vi "GO alerte min-max temperatures.vi"(3 "Numéro":u8) -> (0 "défaut températures min/max":bool)   [LabVIEW 2022 SP3]
uses:
  Enum/Enum s1.ctl
  Variables globales/Variable glob alertes min-max temperatures.vi
  Variables globales/Variable glob mails.vi
  Variables globales/Variables glob EUROTHERM.vi
  Variables globales/Variable glob Th.vi
  Variables globales/Variable glob generale.vi
  Variables globales/Variable glob Pt.vi
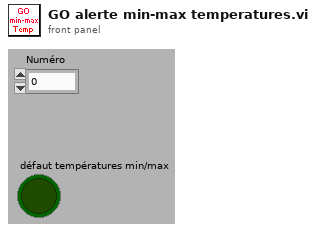
[diagram p1: front panel]
types:
  T1 = typedef "Enum s1.ctl" = enum16{"Alerte vide", "Alerte temperature min-max", "Alerte temperature ecart", "Alerte Keller", "Alerte compteur", "Alerte régulateurs"}
  T2 = cluster{"Alerte temp min/max":bool, "température max":dbl, "température min":dbl, "Défaut min/max temp":bool, "Indices à controler":i16[], "N°":u16}[]
  T3 = cluster{"Alerte temp min/max":bool, "température max":dbl, "température min":dbl, "Défaut min/max temp":bool, "Indices à controler":i16[], "N°":u16}
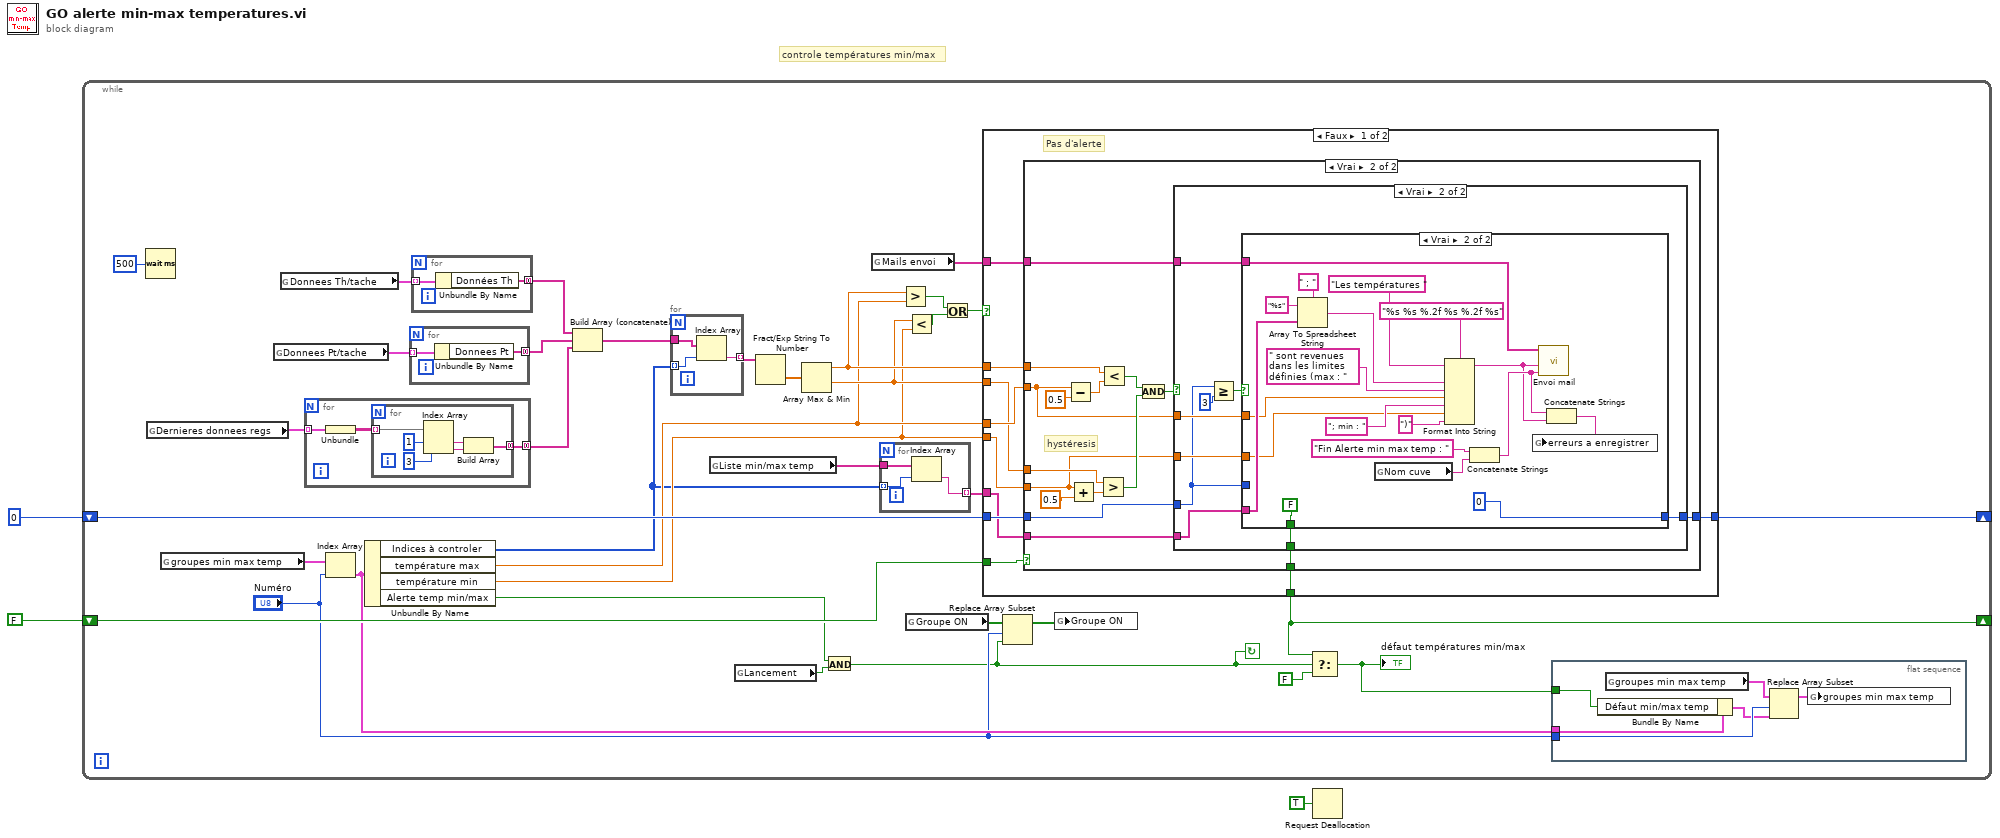
[diagram p0: block diagram]
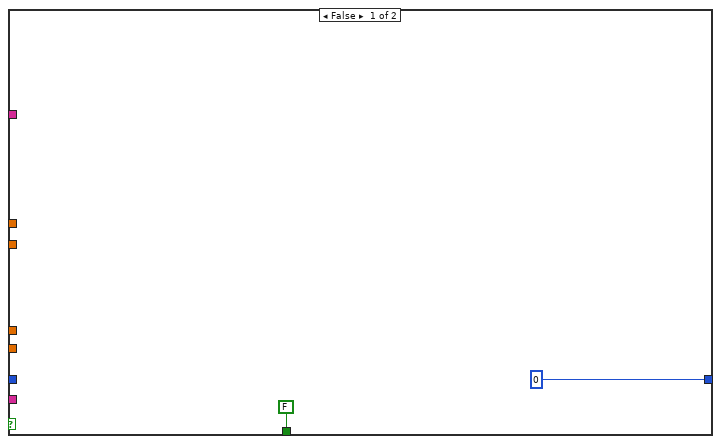
[diagram p2: hidden frame]
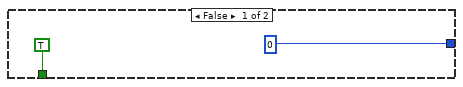
[diagram p3: hidden frame]
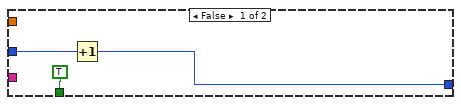
[diagram p4: hidden frame]
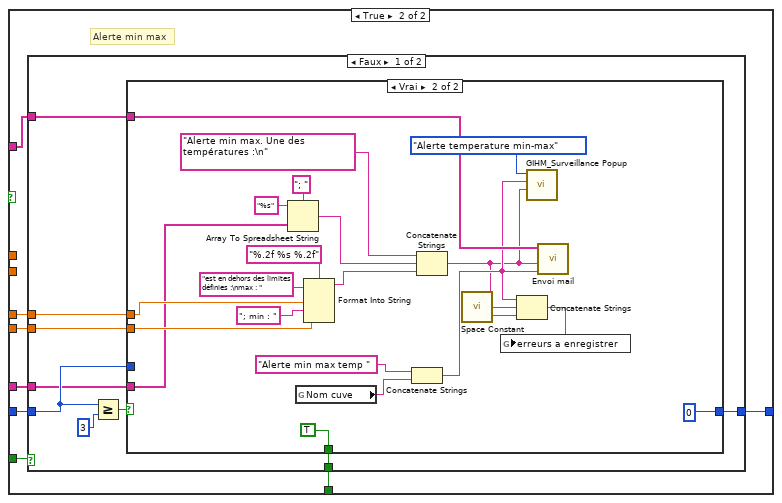
[diagram p5: hidden frame]
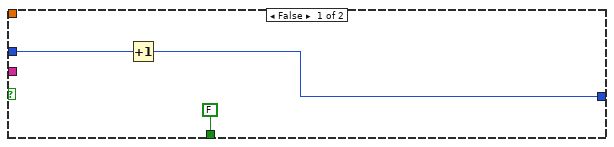
[diagram p6: hidden frame]
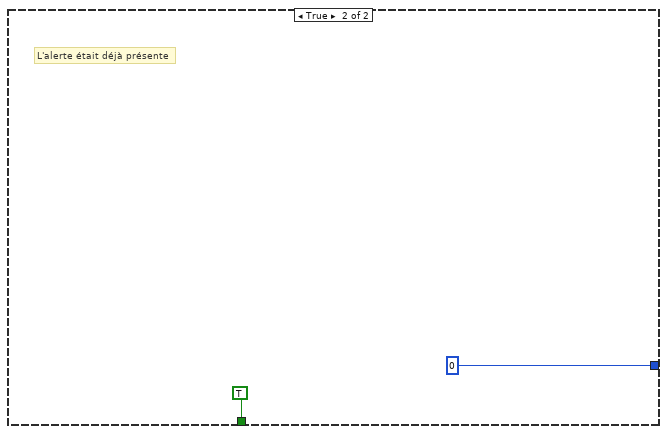
[diagram p7: hidden frame]
diagram:
  # "controle températures min/max"
  n1 = while {
    shift-right: [w22] -> _
    shift-left: FALSE -> [w35]
    shift-right: [w27] -> _
    shift-left: 0 -> [w28]
    stop <- w4 continue-if-true
    n2 = Wait (ms)(milliseconds to wait=u32 500 ("attente (ms)")) -> ()  [unwired: 1 out]
    n3 = global read "Variables glob EUROTHERM.vi" "Dernieres donnees regs"() -> (w18:cluster{"Dernieres donnees 1COM":string[][]}[])
    n4 = global read "Variable glob alertes min-max temperatures.vi" "groupes min max temp"() -> (w13:T2)
    n5 = global read "Variable glob Pt.vi" "Donnees Pt/tache"() -> (w24:cluster{"Donnees Pt":string[]}[])
    n6 = global read "Variable glob Th.vi" "Donnees Th/tache"() -> (w26:cluster{"Données Th":string[]}[])
    n7 = for {
      tunnel: w18 -> [w50] mode=indexing
      tunnel: [w48] -> w17 mode=concatenating
      n8 = Unbundle(w50) -> ("Dernieres donnees 1COM"=w49:string[][])
      n9 = for {
        tunnel: w49 -> [w56] mode=indexing
        tunnel: [w51] -> w48 mode=concatenating
        n10 = Index Array(array=w56, index #1=1 ("indice"), index #2=3 ("longueur")) -> (element #1=w53:string, element #2=w52:string)
        n11 = Build Array(w53, w52) -> (w51:string[])
      }
    }
    n12 = Index Array(array=w13, index="Numéro") -> (element=w15:T3)
    n13 = Unbundle By Name(w15) -> ("Indices à controler"=w12:i16[], "température max"=w20:dbl, "température min"=w19:dbl, "Alerte temp min/max"=w9:bool)
    n14 = for {
      tunnel: w24 -> [w58] mode=indexing
      tunnel: [w57] -> w23 mode=concatenating
      n15 = Unbundle By Name(w58) -> ("Donnees Pt"=w57:string[])
    }
    n16 = for {
      tunnel: w26 -> [w60] mode=indexing
      tunnel: [w59] -> w25 mode=concatenating
      n17 = Unbundle By Name(w60) -> ("Données Th"=w59:string[])
    }
    n18 = Build Array (concatenate)(w25, w23, w17) -> (w31:string[])
    n19 = for {
      tunnel: w31 -> [w166]
      tunnel: w12 -> [w167] mode=indexing
      tunnel: [w165] -> w38 mode=indexing
      n20 = Index Array(array=w166, index=w167) -> (element=w165:string)
    }
    n21 = global read "Variable glob alertes min-max temperatures.vi" "Liste min/max temp"() -> (w11:string[])
    n22 = global read "Variable glob generale.vi" "Lancement"() -> (w33:bool)
    n23 = Fract/Exp String To Number(string=w38) -> (number=w34:dbl[])  [unwired: 3 in, 1 out]
    n24 = Array Max & Min(array=w34) -> (max value=w30:dbl, min value=w29:dbl)  [unwired: 2 out]
    n25 = And(x=w9, y=w33) -> (x .and. y?=w4:bool)
    n26 = global read "Variable glob mails.vi" "Mails envoi"() -> (w8:string[])
    n27 = for {
      tunnel: w12 -> [w46] mode=indexing
      tunnel: w11 -> [w47]
      tunnel: [w45] -> w10 mode=indexing
      n28 = Index Array(array=w47, index=w46) -> (element=w45:string)
    }
    n29 = Greater?(x=w30, y=w20) -> (0:w36:bool)
    n30 = global read "Variable glob alertes min-max temperatures.vi" "Groupe ON"() -> (w7:bool[])
    n31 = Less?(x=w29, y=w19) -> (x < y?=w37:bool)
    n32 = Or(x=w36, y=w37) -> (x .or. y?=w32:bool)
    n33 = case shown="Faux" w32 {
      tunnel: w35 -> [w70 w129]
      tunnel: w8 -> [w69 w128]
      tunnel: w30 -> [w68 _]
      tunnel: w20 -> [w67 w125]
      tunnel: w29 -> [w66 _]
      tunnel: w19 -> [w65 w126]
      tunnel: [w64 w127] -> w22
      tunnel: w28 -> [w63 w124]
      tunnel: [w62 w123] -> w27
      tunnel: w10 -> [w61 w122]
      frame False {
        # "Pas d'alerte"
        # "Pas ou plus d'alerte"
        n34 = case shown="Vrai" w70 {
          tunnel: w69 -> [_ w88]
          tunnel: w68 -> [_ w81]
          tunnel: w67 -> [_ w79]
          tunnel: w66 -> [_ w84]
          tunnel: w65 -> [_ w78]
          tunnel: [FALSE w76] -> w64
          tunnel: w63 -> [_ w74]
          tunnel: [0 w75] -> w62
          tunnel: w61 -> [_ w73]
          frame False {
            # "Il n'y avait pas d'alerte la fois précédente"
          }
          frame True {
            # "hystéresis"
            # "Il y avait une alerte la fois précédente"
            n35 = Subtract(x=w79, y=0.5) -> (x-y=w80:dbl)
            n36 = Add(x=w78, y=0.5) -> (x+y=w85:dbl)
            n37 = Greater?(x=w84, y=w85) -> (0:w82:bool)
            n38 = Less?(x=w81, y=w80) -> (x < y?=w83:bool)
            n39 = And(x=w83, y=w82) -> (x .and. y?=w77:bool)
            n40 = case shown="Vrai" w77 {
              tunnel: w88 -> [_ w99]
              tunnel: w79 -> [_ w98]
              tunnel: w78 -> [_ w97]
              tunnel: [TRUE w92] -> w76
              tunnel: [0 w93] -> w75
              tunnel: w74 -> [_ w94]
              tunnel: w73 -> [_ w91]
              frame False {
              }
              frame True {
                n41 = Greater Or Equal?(x=w94, y=3) -> (x >= y?=w96:bool)
                n42 = case shown="Vrai" w96 {
                  tunnel: w99 -> [_ w121]
                  tunnel: w98 -> [_ w106]
                  tunnel: w97 -> [_ w104]
                  tunnel: w94 -> [w102 _]
                  tunnel: [w101 0] -> w93
                  tunnel: [TRUE FALSE] -> w92
                  tunnel: w91 -> [_ w111]
                  frame False {
                    n43 = Increment(x=w102) -> (x+1=w101:i32)
                  }
                  frame True {
                    n44 = Array To Spreadsheet String(delimiter (Tab)=" ; " ("séparateur (Tabulation)"), array=w111, 3:"%s" ("chaîne de format")) -> (spreadsheet string=w108:string)
                    n45 = global read "Variable glob generale.vi" "Nom cuve"() -> (w117:string)
                    n46 = Format Into String(format string="%s %s %.2f %s %.2f %s" ("chaîne de format"), initial string="Les températures ", w108, " sont revenues dans les limites définies (max : ", w106, "; min : ", w104, ")") -> (resulting string=w112:string)  [unwired: 1 in, 1 out]
                    n47 = Concatenate Strings("Fin Alerte min max temp : " ("subject ([No Subject])"), w117) -> (w113:string)
                    n48 = call "Envoi mail.vi"("Objet"=w113, "Message"=w112, "Mail liste"=w121) -> ()  [unwired: 3 in]
                    n49 = Concatenate Strings(w113, w112) -> (w114:string)
                    n50 = global write "Variable glob generale.vi" "erreurs a enregistrer"(w114) -> ()
                  }
                }
              }
            }
          }
        }
      }
      frame True {
        # "Alerte min max"
        # "Alerte min/max"
        n51 = case shown="Faux" w129 {
          tunnel: w128 -> [w138 _]
          tunnel: [w137 TRUE] -> w127
          tunnel: w126 -> [w135 _]
          tunnel: w125 -> [w136 _]
          tunnel: w124 -> [w131 _]
          tunnel: [w134 0] -> w123
          tunnel: w122 -> [w130 _]
          frame False {
            n52 = Greater Or Equal?(x=w131, y=3) -> (x >= y?=w133:bool)
            n53 = case shown="Vrai" w133 {
              tunnel: w138 -> [_ w161]
              tunnel: [FALSE TRUE] -> w137
              tunnel: w136 -> [_ w154]
              tunnel: w135 -> [_ w153]
              tunnel: [w140 0] -> w134
              tunnel: w131 -> [w141 _]
              tunnel: w130 -> [_ w148]
              frame False {
                n54 = Increment(x=w141) -> (x+1=w140:i32)
              }
              frame True {
                n55 = Array To Spreadsheet String(delimiter (Tab)="; " ("séparateur (Tabulation)"), array=w148, 3:"%s" ("chaîne de format")) -> (spreadsheet string=w156:string)
                n56 = global read "Variable glob generale.vi" "Nom cuve"() -> (w147:string)
                n57 = Format Into String(format string="%.2f %s %.2f" ("chaîne de format"), initial string="est en dehors des limites définies :\nmax : ", w154, "; min : ", w153) -> (resulting string=w151:string)  [unwired: 1 in, 1 out]
                n58 = Concatenate Strings("Alerte min max temp " ("subject ([No Subject])"), w147) -> (w144:string)
                n59 = Concatenate Strings("Alerte min max. Une des températures :\n", w156, w151) -> (w143:string)
                n60 = call <vilib>:"Space Constant.vi"() -> ("String"=w145:string)
                n61 = Concatenate Strings(w144, w145, w143) -> (w146:string)
                n62 = global write "Variable glob generale.vi" "erreurs a enregistrer"(w146) -> ()
                n63 = call "GIHM_Surveillance Popup.vi"("Message"=w143, "Problème observé"=w144, "Type problème"=Enum_s1."Alerte temperature min-max") -> ()  [unwired: 2 in, 1 out]
                n64 = call "Envoi mail.vi"("Objet"=w144, "Message"=w143, "Mail liste"=w161) -> ()  [unwired: 3 in]
              }
            }
          }
          frame True {
            # "L'alerte était déjà présente"
          }
        }
      }
    }
    n65 = Replace Array Subset(array=w7, new element=w4, index="Numéro") -> (w5:bool[])
    n66 = global write "Variable glob alertes min-max temperatures.vi" "Groupe ON"(w5) -> ()
    n67 = Select(t=w22, s=w4, f=FALSE ("cas faux")) -> (s? t:f=w14:bool)
    "défaut températures min/max" <- w14
    n68 = flat-sequence {
      tunnel: w15 -> [w44]
      tunnel: w14 -> [w43]
      tunnel: "Numéro" -> [w42]
      frame #0 {
        n69 = Bundle By Name(cluster=w44, "Défaut min/max temp"=w43) -> (w41:T3)
        n70 = global read "Variable glob alertes min-max temperatures.vi" "groupes min max temp"() -> (w39:T2)
        n71 = Replace Array Subset(array=w39, new element=w41, index=w42) -> (w40:T2)
        n72 = global write "Variable glob alertes min-max temperatures.vi" "groupes min max temp"(w40) -> ()
      }
    }
  }
  n73 = Request Deallocation(TRUE ("flag")) -> ()
